vi "Create_Alarm_Message.vi"(6 "Temperature_Limit":dbl, 7 "Humidity_Limit":dbl, 8 "New_Water_Alarm":bool, 9 "New_Humidity_Alarm":bool, 10 "New_Temperteture_Alarm":bool, 11 "Measurement_Data":T1) -> (2 "SMS_Message":string)   [LabVIEW 2026]
uses:
  Measurement_Data.ctl
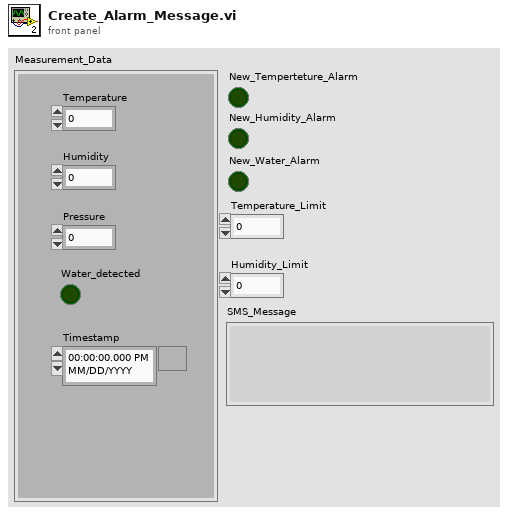
[diagram p1: front panel]
types:
  T1 = typedef "Measurement_Data.ctl" = cluster{"Temperature":dbl, "Humidity":dbl, "Pressure":dbl, "Water_detected":bool, "Timestamp":timestamp}
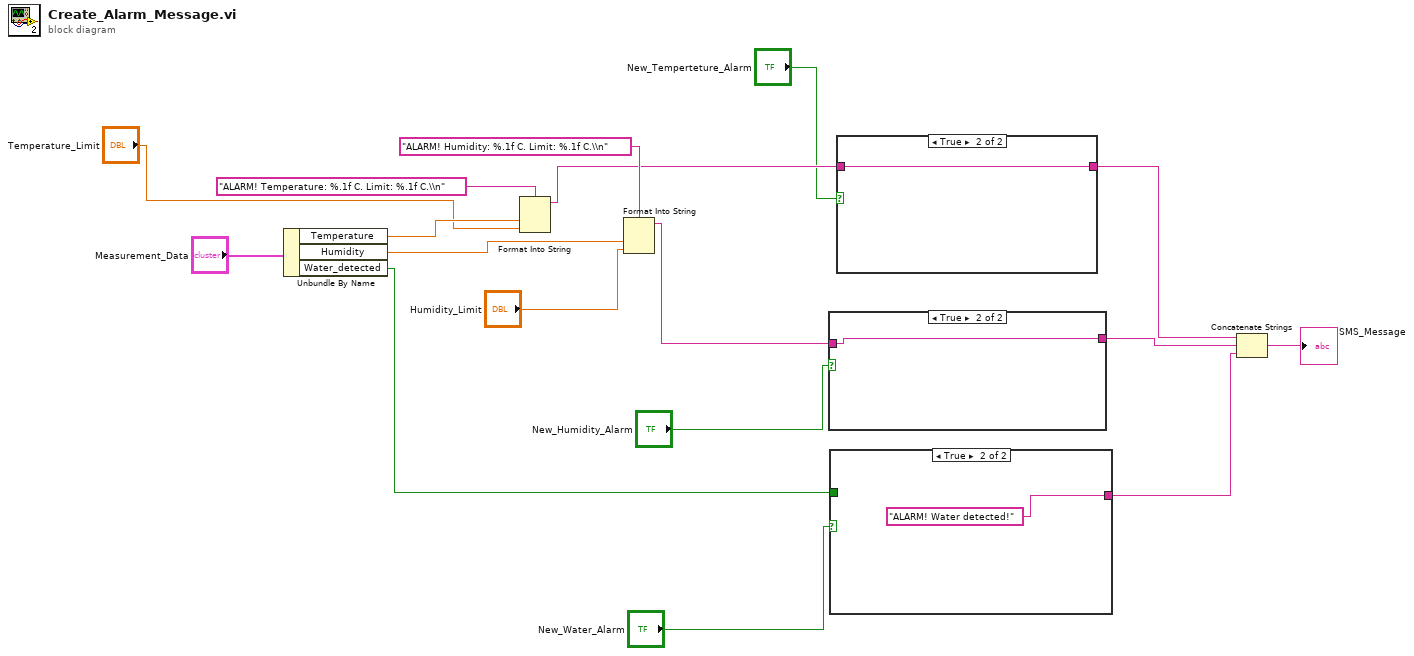
[diagram p0: block diagram]
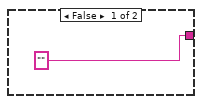
[diagram p2: hidden frame]
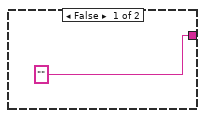
[diagram p3: hidden frame]
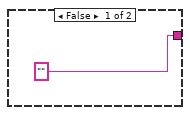
[diagram p4: hidden frame]
diagram:
  n1 = Unbundle By Name("Measurement_Data") -> ("Temperature"=w16:dbl, "Humidity"=w14:dbl, "Water_detected"=w5:bool)
  n2 = Format Into String(format string="ALARM! Temperature: %.1f C. Limit: %.1f C.\\n", w16, "Temperature_Limit") -> (resulting string=w10:string)  [unwired: 2 in, 1 out]
  n3 = Format Into String(format string="ALARM! Humidity: %.1f C. Limit: %.1f C.\\n", w14, "Humidity_Limit") -> (resulting string=w6:string)  [unwired: 2 in, 1 out]
  n4 = case shown="True" "New_Humidity_Alarm" {
    tunnel: w6 -> [_ w19]
    tunnel: ["" w19] -> w3
    frame False {
    }
    frame True {
    }
  }
  n5 = case shown="True" "New_Water_Alarm" {
    tunnel: ["" "ALARM! Water detected!" ("format string")] -> w2
    tunnel: w5 -> [_ _]
    frame False {
    }
    frame True {
    }
  }
  n6 = case shown="True" "New_Temperteture_Alarm" {
    tunnel: w10 -> [_ w23]
    tunnel: ["" w23] -> w4
    frame False {
    }
    frame True {
    }
  }
  n7 = Concatenate Strings(w4, w3, w2) -> (→"SMS_Message":string)
